vi "Example - Simple MQTT client.vi"() -> ()   [LabVIEW 2019]
uses:
  src/KoRE-MQTT.lvlib
  <vilib>/Utility/miscctls.llb/LVRowAndColumnUnsignedTypeDef.ctl
  src/KoRE-MQTT/Public/TypeDefs/MQTT Version.ctl
panel:
  out "Topics:":i32
  out "Last disconnect error or reason:":string
  in  "Client ID":string
  out "Reconnects:":i32
  in  "Pause Update":bool caption="Show data"
  in  "Messages":i32(listbox)
  in  "Subscriptions":T1(array[cluster])
  in  "QoS Level":T2(ring)
  in  "Port":u16=1883
  in  "Host":string(combo)="test.mosquitto.org"
  in  "Password":string
  in  "Username":string
  out "Messages:":u64
  in  "Retain":bool
  in  "Version":T3=4 items=["3.11"=4, "5.0"=5]
  in  "Topic":string
  in  "Send":bool
  in  "Message":string="Message to self!"
  in  "Exit":bool
  # "($SYS/# and a private topic will be added)"
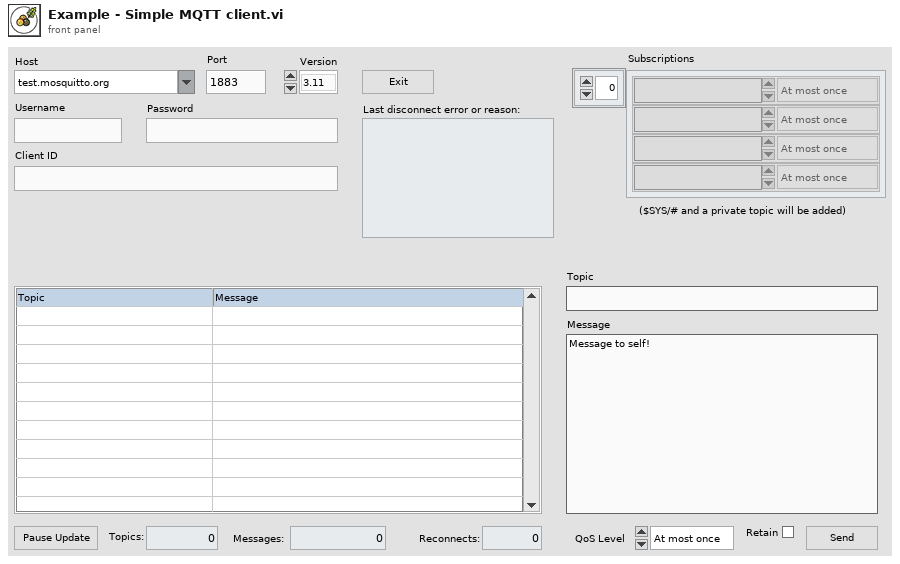
[diagram p1: front panel]
types:
  T1 = cluster{"Topic":string, "QoS":enum16{"At most once", "At least once", "Exactly once"}}[]
  T2 = enum16{"At most once", "At least once", "Exactly once"}
  T3 = typedef "KoRE-MQTT.lvlib/MQTT Version.ctl" = u16
  T4 = typedef "KoRE-MQTT.lvlib/MQTT Refnum.ctl" = refnum<vi>
  T5 = enum8{"Enabled", "Disabled", "Disabled and Grayed Out"}
  T6 = typedef "LVRowAndColumnUnsignedTypeDef.ctl" = cluster{"Row":u32, "Column":u32}
  T7 = cluster{"Topic":string, "QoS":enum16{"At most once", "At least once", "Exactly once"}}
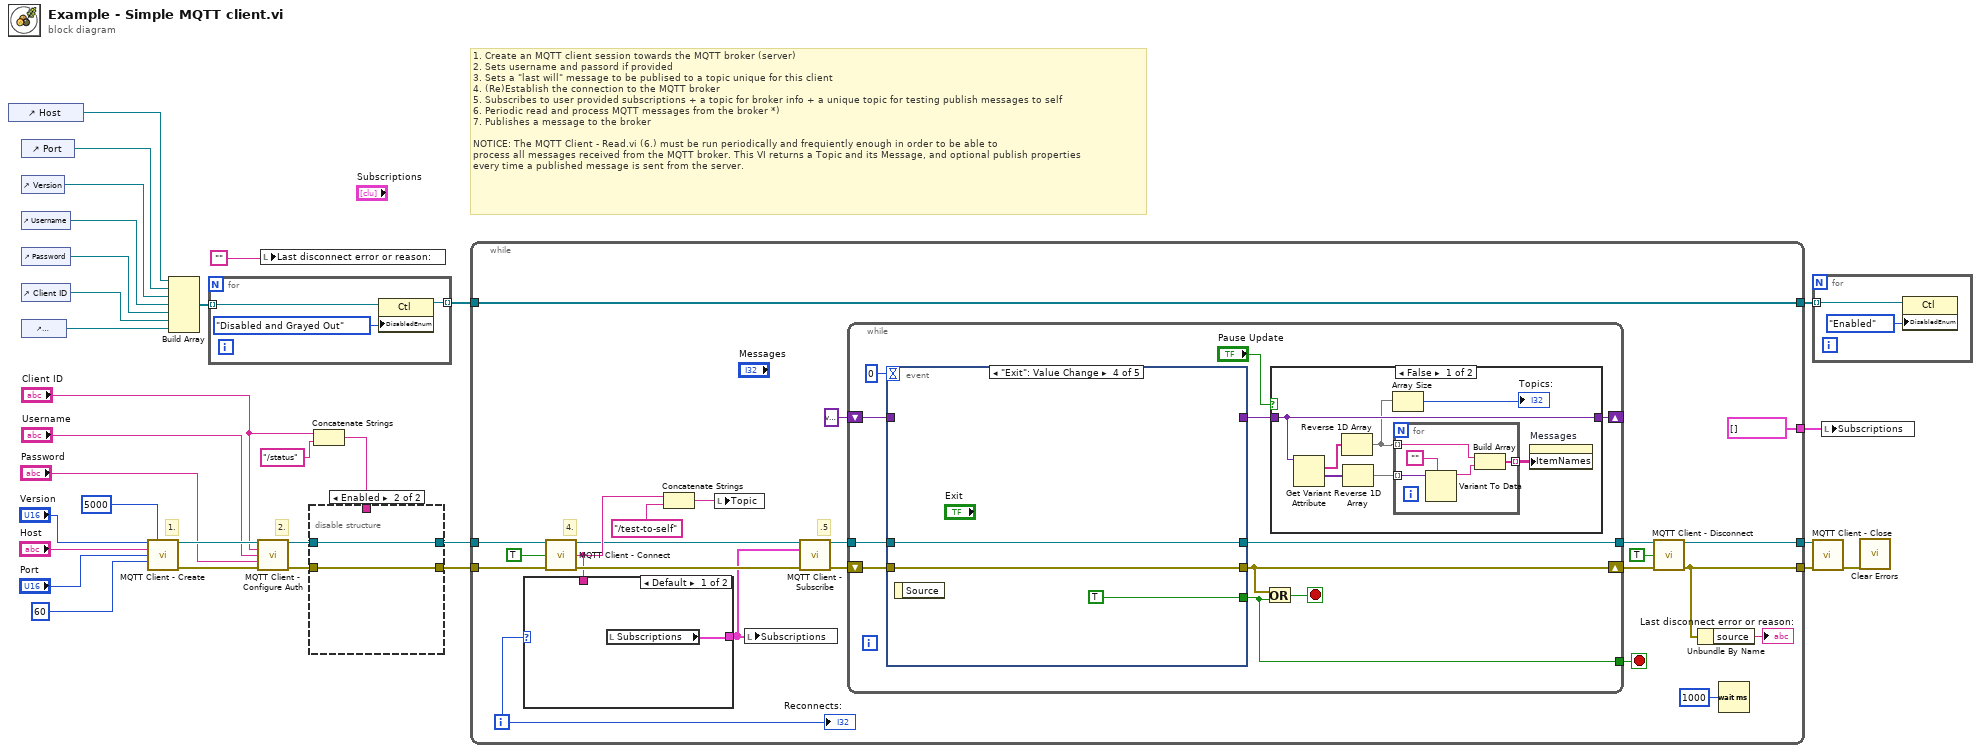
[diagram p0: block diagram]
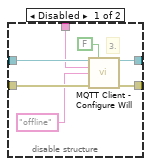
[diagram p2: hidden frame]
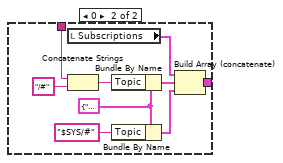
[diagram p3: hidden frame]
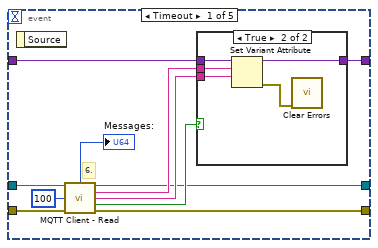
[diagram p4: hidden frame]
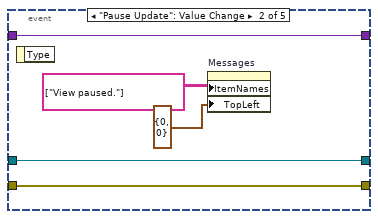
[diagram p6: hidden frame]
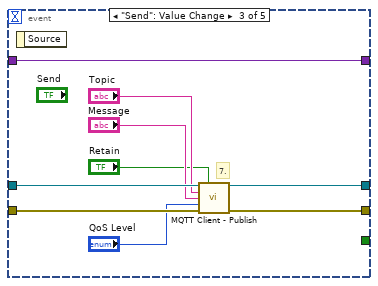
[diagram p7: hidden frame]
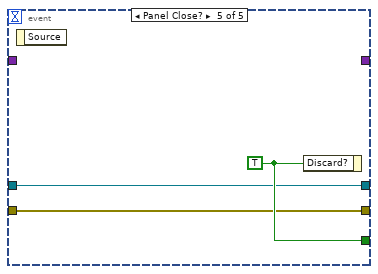
[diagram p8: hidden frame]
diagram:
  # "1. Create an MQTT client session towards the MQTT broker (server)\n2. Sets username and passord if provided\n3. Sets a \"last will\" message to be publised to a topic unique for this client\n4. (Re)Establish the connection to the MQTT broker\n5. Subscribes to user provided subscriptions + a topic for broker info + a unique topic for testing publish messages to self\n6. Periodic read and process MQTT messages from the broker *) \n7. Publishes a message to the broker\n\nNOTICE: The MQTT Client - Read.vi (6.) must be run periodically and frequiently enough in order to be able to\nprocess all messages received from the MQTT broker. This VI returns a Topic and its Message, and optional publish properties\nevery time a published message is sent from the server."
  # "2."
  # "1."
  n1 = control-ref of="Host"() -> (w13:refnum<vi>)
  n2 = control-ref of="Port"() -> (w12:refnum<vi>)
  n3 = control-ref of="Version"() -> (w11:refnum<vi>)
  n4 = control-ref of="Username"() -> (w10:refnum<vi>)
  n5 = control-ref of="Password"() -> (w9:refnum<vi>)
  n6 = control-ref of="Client ID"() -> (w8:refnum<vi>)
  n7 = control-ref of="Subscriptions"() -> (w7:refnum<vi>)
  n8 = call "MQTT Client - Create.vi"("Version (3.11)"="Version", "TCP Timeout (3000 ms)"=5000 ("TCP Timeout (ms)"), "Host"="Host", "Port (1883)"="Port", "Keep Alive (60 s)"=u16 60 ("Keep Alive s (60)")) -> ("MQTT Session"=w29:T4, "error out"=w28:errorcluster)  [unwired: 9 in]
  n9 = Build Array(w13, w12, w11, w10, w9, w8, w7) -> (w6:refnum<vi>[])
  n10 = for {
    tunnel: w6 -> [w34] mode=indexing
    tunnel: [w32] -> w5 mode=indexing
    n11 = property class="Ctl"(reference=w34, "DisabledEnum"=T5."Disabled and Grayed Out" ("Disabled")) -> (reference out=w32:refnum<vi>)  [unwired: 1 in, 1 out]
  }
  n12 = call "MQTT Client - Configure Auth.vi"("MQTT Session"=w29, "Client ID"="Client ID", "Username"="Username", "Password"="Password", "error in (no error)"=w28) -> ("MQTT Session out"=w21:T4, "error out"=w22:errorcluster)  [unwired: 9 in]
  n13 = local write "Last disconnect error or reason:"("") -> ()
  n14 = Concatenate Strings("Client ID", "/status" ("string")) -> (w20:string)
  n15 = disable-structure shown="Enabled" {
    disable-tunnel: w22 -> [w41 w42]
    disable-tunnel: w21 -> [w40 w43]
    disable-tunnel: w20 -> [w39 _]
    disable-tunnel: [w36 w43] -> w15
    disable-tunnel: [w35 w42] -> w14
    frame Disabled {
      # "3."
      n16 = call "MQTT Client - Configure Will.vi"("MQTT Session"=w40, "Will Retain (False)"=FALSE ("Will Retain"), "Will Topic"=w39, "Will Payload"="offline", "error in"=w41) -> ("MQTT Session out"=w36:T4, "error out"=w35:errorcluster)  [unwired: 9 in]
    }
    frame Enabled {
    }
  }
  n17 = while {
    tunnel: w14 -> [w65]
    tunnel: w15 -> [w45]
    tunnel: [w58] -> w31
    tunnel: [w56] -> w30
    tunnel: [w54] -> w4
    tunnel: w5 -> [w54]
    tunnel: [T1 [] ("Subscriptions")] -> w2
    i -> [w46]
    stop <- w61 stop-if-true
    # ".5"
    # "4."
    n18 = call "MQTT Client - Connect.vi"("MQTT Session"=w45, "Clean Start"=TRUE, "error in (no error)"=w65) -> ("MQTT Session out"=w44:T4, "Assigned Client Identifier"=w53:string, "error out"=w66:errorcluster)  [unwired: 8 in, 2 out]
    n19 = case shown="Default" w46 {
      tunnel: w53 -> [_ w72]
      tunnel: [w67 w71] -> w50
      frame Default {
        n20 = local read "Subscriptions"() -> (w67:T1)
      }
      frame 0 {
        w70 = T7 {"Topic"="", "QoS"=enum."At most once"} ("QoS")
        n21 = local read "Subscriptions"() -> (w73:T1)
        n22 = Concatenate Strings(w72, "/#" ("string")) -> (w75:string)
        n23 = Bundle By Name(cluster=w70, "Topic"=w75) -> (w76:T7)
        n24 = Bundle By Name(cluster=w70, "Topic"="$SYS/#") -> (w69:T7)
        n25 = Build Array (concatenate)(w73, w76, w69) -> (w71:T1)
      }
    }
    n26 = Concatenate Strings(w53, "/test-to-self" ("string")) -> (w51:string)
    n27 = local write "Topic"(w51) -> ()
    n28 = local write "Subscriptions"(w50) -> ()
    n29 = call "MQTT Client - Subscribe.vi"("MQTT Session"=w44, "Multiple Topics"=w50, "error in (no error)"=w66) -> ("MQTT Session out"=w63:T4, "error out"=w60:errorcluster)  [unwired: 11 in]
    n30 = while {
      shift-right: [w80] -> w48
      shift-left: w60 -> [w87]
      tunnel: w63 -> [w86]
      shift-right: [w81] -> _
      shift-left: variant -> [w84]
      tunnel: [w78] -> w59
      tunnel: [w77] -> w61
      stop <- w79 stop-if-true
      n31 = event shown="[3] \"Exit\": Value Change" {
        selector: _ -> [_ _ _ _ _]
        dyn-events: _ -> [_ _ _ _ _]
        timeout: 0 -> [_ _ _ _ _]
        tunnel: w87 -> [w98 w106 w118 w120 w123]
        tunnel: w86 -> [w96 w105 w116 w119 w122]
        tunnel: [w97 w106 w117 w120 w123] -> w80
        tunnel: [_ _ _ TRUE w124] -> w77
        tunnel: [w93 w107 w113 _ _] -> w82
        tunnel: w84 -> [w92 w107 w113 _ _]
        tunnel: [w90 w105 w112 w119 w122] -> w78
        event Timeout {
          # "6."
          n32 = event-data() -> ()  [unwired: 1 in, 1 out]
          n33 = call "MQTT Client - Read.vi"("MQTT Session"=w96, "timeout (global)"=100, "error in (no error)"=w98) -> ("# received"=→"Messages:":u64, "MQTT Session out"=w90:T4, "Topic"=w95:string, "Message"=w94:string, "New message?"=w91:bool, "error out"=w97:errorcluster)  [unwired: 6 in, 1 out]
          n34 = case shown="True" w91 {
            tunnel: w95 -> [_ w104]
            tunnel: w94 -> [_ w103]
            tunnel: [w99 w102] -> w93
            tunnel: w92 -> [w99 w101]
            frame False {
            }
            frame True {
              n35 = Set Variant Attribute(Variant=w101, name=w104, value=w103) -> (Variant out=w102:variant, error out=w100:errorcluster)  [unwired: 1 in, 1 out]
              n36 = call <vilib>:"Clear Errors.vi"("error in (no error)"=w100) -> ()  [unwired: 5 in, 2 out]
            }
          }
        }
        event "Pause Update": Value Change {
          n37 = event-data() -> ()  [unwired: 1 in, 1 out]
          n38 = property on="Messages" class="MCListbox (strict)"("ItemNames"=string[][] [["View paused."]], "TopLeft"=T6 {"Row"=0, "Column"=0} ("Top Left Visible Cell")) -> ()  [unwired: 2 in, 2 out]
        }
        event "Send": Value Change {
          # "7."
          n39 = event-data() -> ()  [unwired: 1 in, 1 out]
          n40 = call "MQTT Client - Publish.vi"("MQTT Session"=w116, "Retain"="Retain", "Topic"="Topic", "Message"="Message", "QoS"="QoS Level", "error in"=w118) -> ("MQTT Session out"=w112:T4, "error out"=w117:errorcluster)  [unwired: 8 in]
        }
        event "Exit": Value Change {
          n41 = event-data() -> ()  [unwired: 1 in, 1 out]
        }
        event Panel Close? {
          w124 = TRUE
          n42 = event-data() -> ()  [unwired: 1 in, 1 out]
          n43 = event-data("Discard?"=w124) -> ()  [unwired: 1 in, 1 out]
        }
      }
      n44 = Or(x=w80, y=w77) -> (x .or. y?=w79:bool)
      n45 = case shown="False" "Pause Update" {
        tunnel: w82 -> [w131 w137]
        tunnel: [w131 w137] -> w81
        frame False {
          n46 = Get Variant Attribute(Variant=w131) -> (names=w126:string[], values=w128:variant[])  [unwired: 3 in, 2 out]
          n47 = Reverse 1D Array(array=w126) -> (reversed array=w125:string[])
          n48 = Reverse 1D Array(array=w128) -> (reversed array=w127:variant[])
          n49 = Array Size(array=w125) -> (size(s)=→"Topics:":i32)
          n50 = for {
            tunnel: w125 -> [w134] mode=indexing
            tunnel: w127 -> [w136] mode=indexing
            tunnel: [w132] -> w129 mode=indexing
            n51 = Variant To Data(type="", Variant=w136) -> (data=w133:string)  [unwired: 1 in, 1 out]
            n52 = Build Array(w134, w133) -> (w132:string[])
          }
          n53 = property on="Messages" class="MCListbox (strict)"("ItemNames"=w129) -> ()  [unwired: 2 in, 2 out]
        }
        frame True {
        }
      }
    }
    n54 = call "MQTT Client - Disconnect.vi"("MQTT Session"=w59, "With Will (v5)"=TRUE ("With Will"), "error in (no error)"=w48) -> ("MQTT Session out"=w58:T4, "error out"=w56:errorcluster)  [unwired: 11 in]
    n55 = Unbundle By Name(w56) -> ("source"=→"Last disconnect error or reason:":string)
    n56 = Wait (ms)(milliseconds to wait=u32 1000) -> ()  [unwired: 1 out]
    "Reconnects:" <- w46
  }
  n57 = for {
    tunnel: w4 -> [w139] mode=indexing
    n58 = property class="Ctl"(reference=w139, "DisabledEnum"=T5."Enabled" ("Disabled")) -> ()  [unwired: 1 in, 2 out]
  }
  n59 = call "MQTT Client - Close.vi"("MQTT session"=w31, "error in (no error)"=w30) -> ("error out"=w1:errorcluster)  [unwired: 13 in]
  n60 = local write "Subscriptions"(w2) -> ()
  n61 = call <vilib>:"Clear Errors.vi"("error in (no error)"=w1) -> ()  [unwired: 5 in, 2 out]
